vi "[ex ce] Simple chart of function.vi"() -> ()   [LabVIEW 2021]
doc: "This simplest example evaluates a formula and displays result in a chart.\n\n::: CalcExpress Toolkit :::\nCopyright (c) 2000-2026 Konstantin Shifershteyn. All rights reserved."
panel:
  in  "update period, ms":u32=5
  in  "stop":bool
  out "chart":dbl(graph)
  in  "Expression":string="y = sin(x) + sin(x/3) + sin(x/5);\nx += 0.1;\ny"
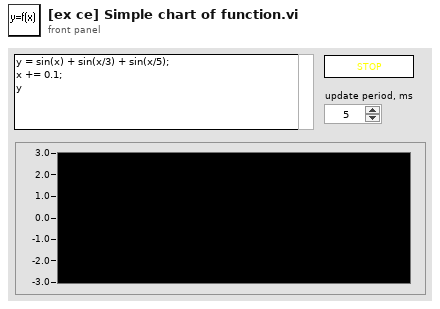
[diagram p1: front panel]
types:
  T1 = enum16{"create", "destroy", "set value", "get value"}
  T2 = typedef "VarMan Variable Context Handle.ctl" = i32
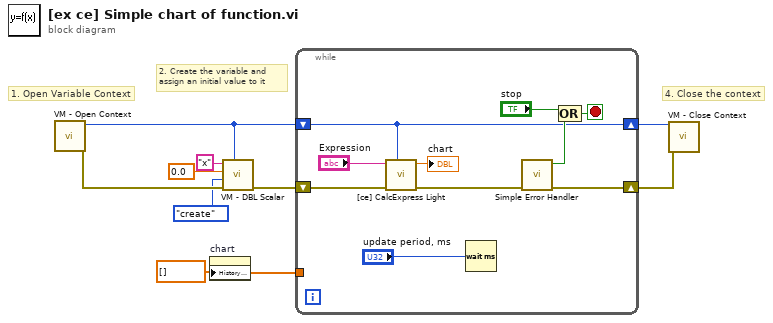
[diagram p0: block diagram]
diagram:
  w7 = dbl[] [] ("History Data")
  # "4. Close the context"
  # "2. Create the variable and\nassign an initial value to it"
  # "1. Open Variable Context"
  n1 = call "VM - Open Context.vi"() -> ("error out"=w8:errorcluster, "VC Handle out"=w1:T2)  [unwired: 9 in, 1 out]
  n2 = property on="chart" class="WFChart (strict)"("History Data"=w7) -> ()  [unwired: 2 in, 2 out]
  n3 = call "VM - DBL Scalar.vi"("VC Handle"=w1, "error in"=w8, "cmd"=T1."create", "value in"=0.0 ("value (0)"), "name_spec"="x" ("name")) -> ("error out"=w4:errorcluster)  [unwired: 1 in, 5 out]
  n4 = while {
    tunnel: w7 -> [_]
    shift-right: [w13] -> w3
    shift-left: w4 -> [w10]
    shift-right: [w11] -> w2
    shift-left: w1 -> [w11]
    stop <- w18 stop-if-true
    n5 = call "[ce] CalcExpress Light.vi"("VC Handle"=w11, "error in"=w10, "expression"="Expression") -> ("error out"=w15:errorcluster, "numeric value"=→"chart":dbl)  [unwired: 6 in, 1 out]
    n6 = Wait (ms)(milliseconds to wait="update period, ms") -> ()  [unwired: 1 out]
    n7 = call <vilib>:"Simple Error Handler.vi"("error in (no error)"=w15) -> ("error?"=w14:bool, "error out"=w13:errorcluster)  [unwired: 4 in, 3 out]
    n8 = Compound Arithmetic op=OR("stop", w14) -> (w18:bool)
  }
  n9 = call "VM - Close Context.vi"("error in"=w3, "VC Handle"=w2) -> ()  [unwired: 8 in, 2 out]
